vi "Selected folder_list.vi"(8 "selection":enum16{"10k", "100k"}(ring), 11 "Folder_List":string[](array[string])) -> (3 "selected Folder List":string[](array[string]))   [LabVIEW 2018]
panel:
  out "Array":bool[](array[boolean])
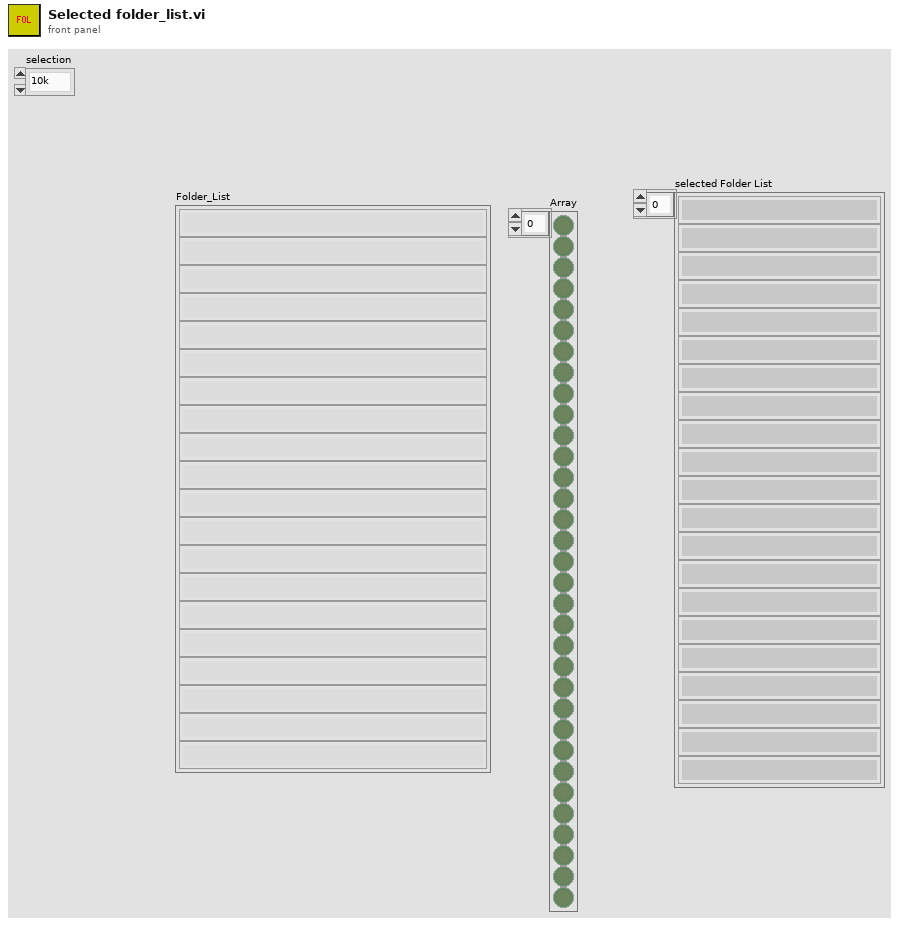
[diagram p1: front panel]
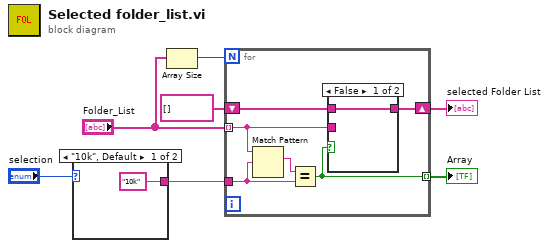
[diagram p0: block diagram]
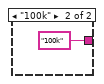
[diagram p2: hidden frame]
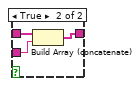
[diagram p3: hidden frame]
diagram:
  n1 = case shown="\"10k\", Default" "selection" {
    tunnel: ["10k" ("search string") "100k" ("search string")] -> w4
    frame "10k", Default {
    }
    frame "100k" {
    }
  }
  n2 = Array Size(array="Folder_List") -> (size(s)=w7:i32)
  n3 = for {
    N: w7 -> [_]
    tunnel: "Folder_List" -> [w12] mode=indexing
    tunnel: [w13] -> w5 mode=indexing
    tunnel: w4 -> [w14]
    shift-right: [w11] -> w2
    shift-left: string[] [] -> [w10]
    n4 = Match Pattern(string=w12, regular expression=w14) -> (match substring=w15:string)  [unwired: 1 in, 3 out]
    n5 = Equal?(x=w15, y=w14) -> (x = y?=w13:bool)
    n6 = case shown="False" w13 {
      tunnel: w12 -> [_ w19]
      tunnel: [w16 w18] -> w11
      tunnel: w10 -> [w16 w17]
      frame False {
      }
      frame True {
        n7 = Build Array (concatenate)(w17, w19) -> (w18:string[])
      }
    }
  }
  "Array" <- w5
  "selected Folder List" <- w2
